vi "[ex ce] Show Waveform graphs.vi"() -> ()   [LabVIEW 2021]
doc: "<B>Example for CalcExpress script syntax</B>\n\nThis simplest example computes some formulas and displays them in a probe window with Waveform Graph. It uses <B>polymorphism</B> of CalcExpress operators and functions to perform computation.\n\n::: CalcExpress Toolkit :::\nCopyright (c) 2000-2026 Konstantin Shifershteyn. All rights reserved."
panel:
  in  "Expression":string="// Initializing of variables\nlowX = pi(-6);\nhigX = pi(6);\ndX = rad(1);\n\n/* create array with values from lowX to higX with step dX */\nX  = nvecifs(lowX, higX, dX);\n\n/* Computing of the formulas */\nY  = 10 * sinc(X);\ndY = derivate(Y, dX, 0,0);\niY = integral(Y, dX, 0,0) / 5;\n\n/* Building of Graphs */\nWFGraph();    // clear graph\nWFGraph(0,  Y, lowX,dX, \"Y=10*Sinc(X)\");\nWFGraph(1, dY, lowX,dX, \"Derivate(Y)\");\nWFGraph(2, iY, lowX,dX, \"Integral(Y)/5\");\n"
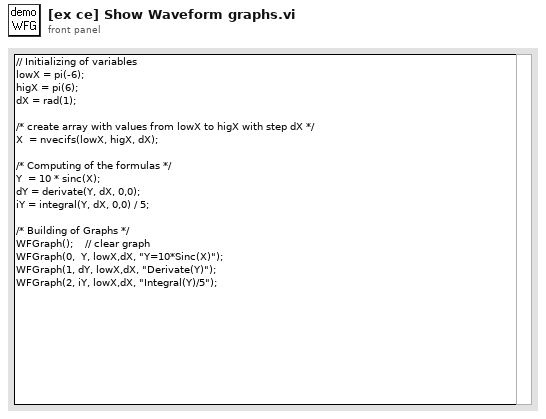
[diagram p1: front panel]
types:
  T1 = typedef "VarMan Variable Context Handle.ctl" = i32
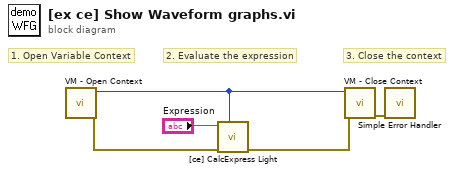
[diagram p0: block diagram]
diagram:
  # "3. Close the context"
  # "2. Evaluate the expression"
  # "1. Open Variable Context"
  n1 = call "VM - Open Context.vi"() -> ("error out"=w5:errorcluster, "VC Handle out"=w1:T1)  [unwired: 9 in, 1 out]
  n2 = call "[ce] CalcExpress Light.vi"("VC Handle"=w1, "error in"=w5, "expression"="Expression") -> ("error out"=w4:errorcluster)  [unwired: 6 in, 2 out]
  n3 = call "VM - Close Context.vi"("error in"=w4, "VC Handle"=w1) -> ("error out"=w3:errorcluster)  [unwired: 8 in, 1 out]
  n4 = call <vilib>:"Simple Error Handler.vi"("error in (no error)"=w3) -> ()  [unwired: 4 in, 5 out]
